vi "Display Error.vi"(2 "Error Type":T1(ring)=enum."Label Error", 7 "Errors":string[](array[string])) -> ()   [LabVIEW 2023]
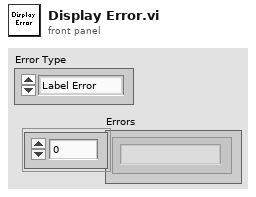
[diagram p1: front panel]
types:
  T1 = enum16{"Channel Error", "Label Error", "Octal Error"}
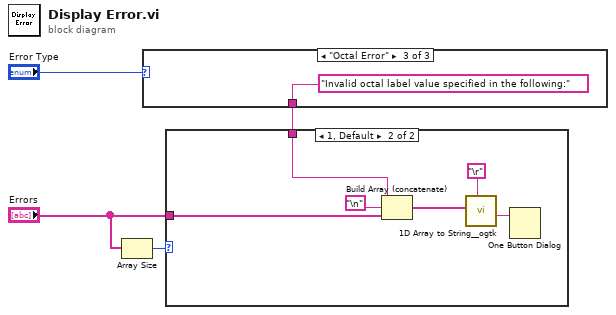
[diagram p0: block diagram]
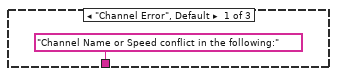
[diagram p2: hidden frame]
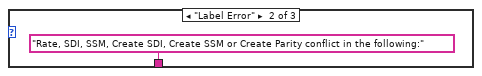
[diagram p3: hidden frame]
diagram:
  n1 = Array Size(array="Errors") -> (size(s)=w3:i32)
  n2 = case shown="\"Octal Error\"" "Error Type" {
    tunnel: ["Channel Name or Speed conflict in the following:" ("string") "Rate, SDI, SSM, Create SDI, Create SSM or Create Parity conflict in the following:" ("string") "Invalid octal label value specified in the following:" ("string")] -> w1
    frame "Channel Error", Default {
    }
    frame "Label Error" {
    }
    frame "Octal Error" {
    }
  }
  n3 = case shown="1, Default" w3 {
    tunnel: "Errors" -> [_ w9]
    tunnel: w1 -> [_ w8]
    frame 0 {
    }
    frame 1, Default {
      n4 = Build Array (concatenate)(w8, "\n", w9) -> (w11:string[])
      n5 = call <userlib>:"1D Array to String__ogtk.vi"("delimiter (Tab)"="\r", "Array of Strings"=w11) -> ("delimited string"=w12:string)  [unwired: 9 in]
      n6 = One Button Dialog(message=w12) -> ()  [unwired: 1 in, 1 out]
    }
  }
